vi "ReadExcelLine.vi"(8 "references":T1, 9 "previous setting":T2, 10 "measurement settings":string[][](array[string]), 11 "row number":i32) -> (0 "references out":T1, 1 "same range?":bool, 3 "measurement setting":T2)   [LabVIEW 2011]
doc: "Parse an row red from the excel template and returnes measurement settings."
uses:
  Measurement Setting.ctl
  Measurement References.ctl
  <vilib>/Utility/NIReport.llb/NI_report.lvclass
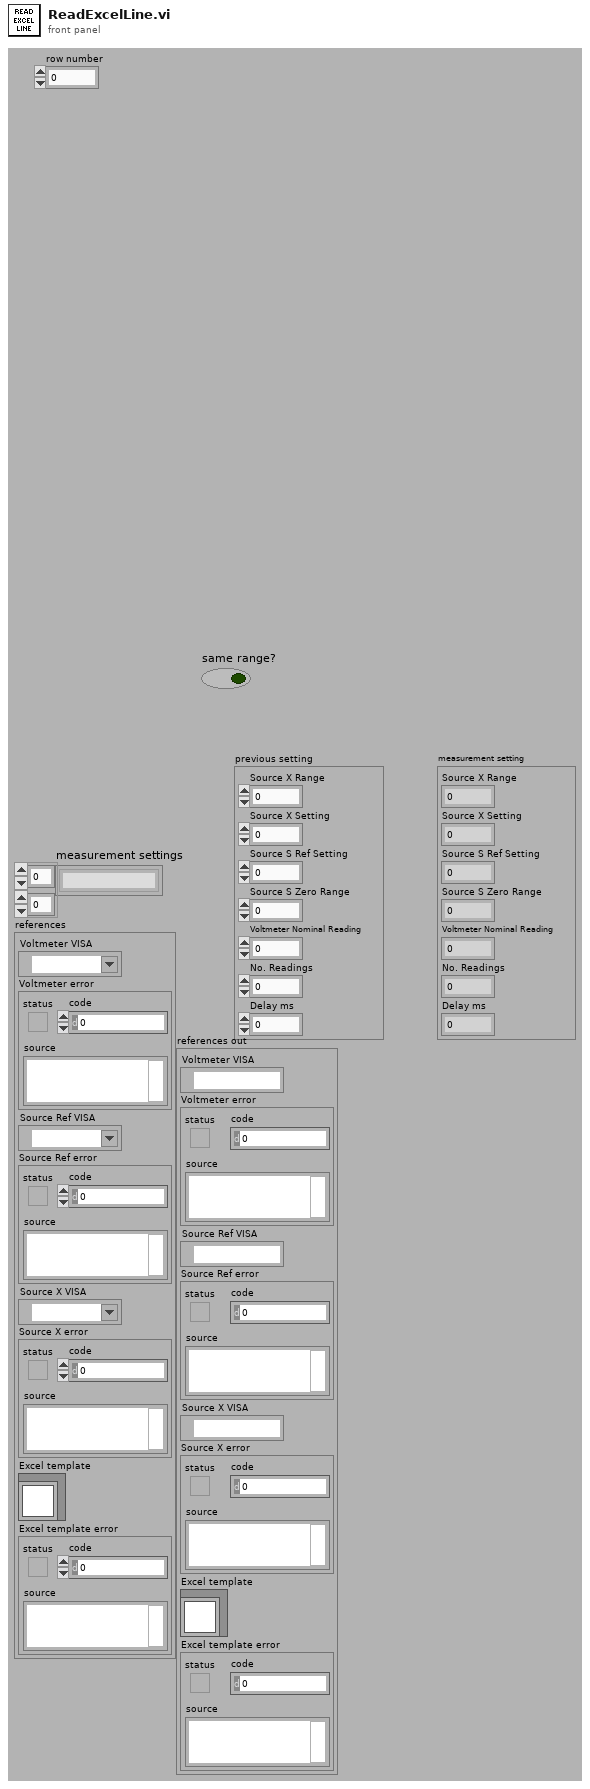
[diagram p1: front panel]
types:
  T1 = typedef "Measurement References.ctl" = cluster{"Voltmeter VISA":refnum<visa-resource-name>, "Voltmeter error":errorcluster, "Source Ref VISA":refnum<visa-resource-name>, "Source Ref error":errorcluster, "Source X VISA":refnum<visa-resource-name>, "Source X error":errorcluster, "Excel template":refnum<class "NI_report.lvclass">, "Excel template error":errorcluster}
  T2 = typedef "Measurement Setting.ctl" = cluster{"Source X Range":dbl, "Source X Setting":dbl, "Source S Ref Setting":dbl, "Source S Zero Range":dbl, "Voltmeter Nominal Reading":dbl, "No. Readings":dbl, "Delay ms":dbl}
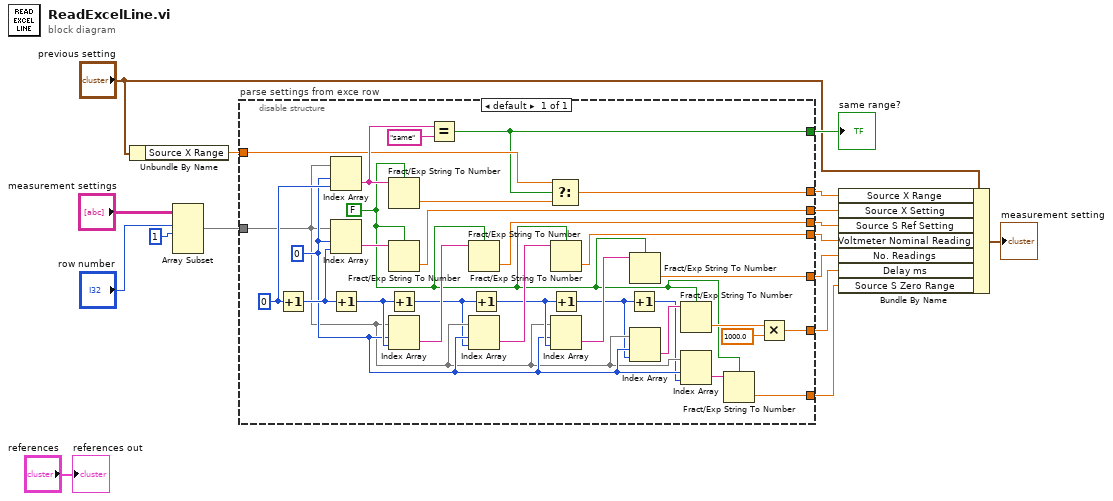
[diagram p0: block diagram]
diagram:
  n1 = Unbundle By Name("previous setting") -> ("Source X Range"=w5:dbl)
  n2 = Array Subset(array="measurement settings", index (row)="row number", length (row)=1 ("length")) -> (w16:string[][])  [unwired: 2 in]
  n3 = disable-structure "parse settings from exce row" shown="default" {
    disable-tunnel: [w46] -> w6
    disable-tunnel: [w43] -> w7
    disable-tunnel: [w42] -> w8
    disable-tunnel: [w41] -> w9
    disable-tunnel: [w40] -> w10
    disable-tunnel: w16 -> [w22]
    disable-tunnel: [w34] -> w11
    disable-tunnel: w5 -> [w26]
    disable-tunnel: [w25] -> w14
    disable-tunnel: [w20] -> w4
    frame Enabled {
      w21 = FALSE ("use system decimal point (T)")
      w24 = 0 ("disabled index (col)")
      w28 = 0 ("index (row)")
      n4 = Increment(x=w28) -> (x+1=w29:i32)
      n5 = Index Array(array=w22, index (row)=w24, index (col)=w28) -> (element=w33:string)
      n6 = Index Array(array=w22, index (row)=w24, index (col)=w29) -> (element=w39:string)
      n7 = Increment(x=w29) -> (x+1=w30:i32)
      n8 = Fract/Exp String To Number(use system decimal point (T)=w21, string=w33) -> (number=w27:dbl)  [unwired: 2 in, 1 out]
      n9 = Fract/Exp String To Number(use system decimal point (T)=w21, string=w39) -> (number=w40:dbl)  [unwired: 2 in, 1 out]
      n10 = Increment(x=w30) -> (x+1=w19:i32)
      n11 = Index Array(array=w22, index (row)=w24, index (col)=w30) -> (element=w38:string)
      n12 = Equal?(x=w33, y="same") -> (x = y?=w25:bool)
      n13 = Fract/Exp String To Number(use system decimal point (T)=w21, string=w38) -> (number=w41:dbl)  [unwired: 2 in, 1 out]
      n14 = Index Array(array=w22, index (row)=w24, index (col)=w19) -> (element=w37:string)
      n15 = Increment(x=w19) -> (x+1=w31:i32)
      n16 = Select(t=w26, s=w25, f=w27) -> (s? t:f=w34:dbl)
      n17 = Fract/Exp String To Number(use system decimal point (T)=w21, string=w37) -> (number=w42:dbl)  [unwired: 2 in, 1 out]
      n18 = Increment(x=w31) -> (x+1=w18:i32)
      n19 = Index Array(array=w22, index (row)=w24, index (col)=w31) -> (element=w36:string)
      n20 = Increment(x=w18) -> (x+1=w17:i32)
      n21 = Fract/Exp String To Number(use system decimal point (T)=w21, string=w36) -> (number=w43:dbl)  [unwired: 2 in, 1 out]
      n22 = Index Array(array=w22, index (row)=w24, index (col)=w18) -> (element=w35:string)
      n23 = Fract/Exp String To Number(use system decimal point (T)=w21, string=w35) -> (number=w45:dbl)  [unwired: 2 in, 1 out]
      n24 = Index Array(array=w22, index (row)=w24, index (col)=w17) -> (element=w23:string)
      n25 = Fract/Exp String To Number(use system decimal point (T)=w21, string=w23) -> (number=w20:dbl)  [unwired: 2 in, 1 out]
      n26 = Multiply(x=w45, y=1000.0) -> (x*y=w46:dbl)
    }
  }
  "same range?" <- w14
  n27 = Bundle By Name(cluster="previous setting", "Source X Range"=w11, "Source X Setting"=w10, "Source S Ref Setting"=w9, "Voltmeter Nominal Reading"=w8, "No. Readings"=w7, "Delay ms"=w6, "Source S Zero Range"=w4) -> (→"measurement setting":T2)
  "references out" <- "references"
